vi "ms_toeplitz.vi"(4 "error in (no error)":errorcluster, 6 "column":cdb[](array[numeric]), 7 "row":cdb[](array[numeric])) -> (0 "error out":errorcluster, 3 "Toeplitz Array":cdb[][](array[numeric]))   [LabVIEW 2026]
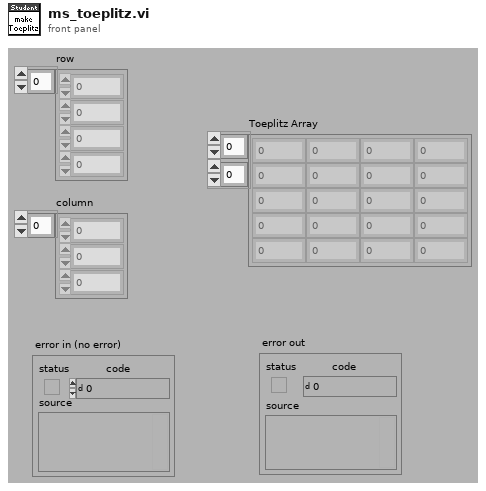
[diagram p1: front panel]
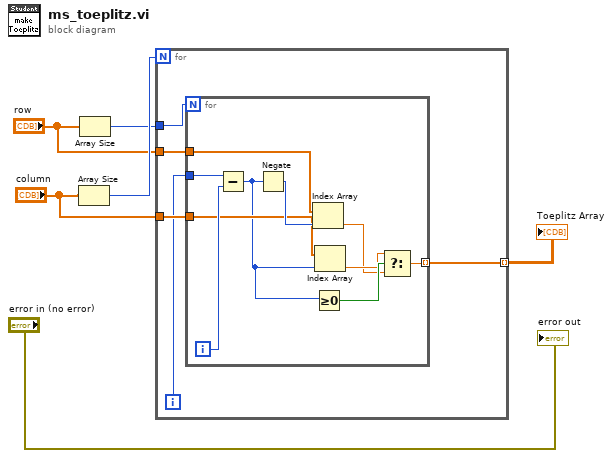
[diagram p0: block diagram]
diagram:
  n1 = Array Size(array="column") -> (size(s)=w6:i32)
  n2 = Array Size(array="row") -> (size(s)=w5:i32)
  n3 = for {
    N: w6 -> [_]
    tunnel: w5 -> [w11]
    tunnel: "row" -> [w10]
    tunnel: "column" -> [w9]
    tunnel: [w7] -> w2 mode=indexing
    i -> [w8]
    n4 = for {
      N: w11 -> [_]
      tunnel: w10 -> [w18]
      tunnel: w9 -> [w17]
      tunnel: w8 -> [w21]
      tunnel: [w12] -> w7 mode=indexing
      i -> [w20]
      n5 = Subtract(x=w21, y=w20) -> (x-y=w16:i32)
      n6 = Negate(x=w16) -> (-x=w19:i32)
      n7 = Index Array(array=w18, index=w19) -> (element=w13:cdb)
      n8 = Greater Or Equal To 0?(x=w16) -> (x >= 0?=w15:bool)
      n9 = Index Array(array=w17, index=w16) -> (element=w14:cdb)
      n10 = Select(t=w14, s=w15, f=w13) -> (s? t:f=w12:cdb)
    }
  }
  "Toeplitz Array" <- w2
  "error out" <- "error in (no error)"
